vi "Project Save As.vi"(8 "error in (no error)":errorcluster, 9 "Rename Paths[]":T1[](array[typedef]), 10 "Existing Project Path":path, 11 "New Project Path":path) -> (0 "error out":errorcluster)   [LabVIEW 2016, in "SLL Scripting.lvlib"]
doc: "Make a copy of the project and rename some of the components of the project including their relinking."
uses:
  SLL Scripting.lvlib
  _Typedefs/Rename Item Cluster.ctl
  <vilib>/Utility/EditLVProj/Edit LVProj.lvlib
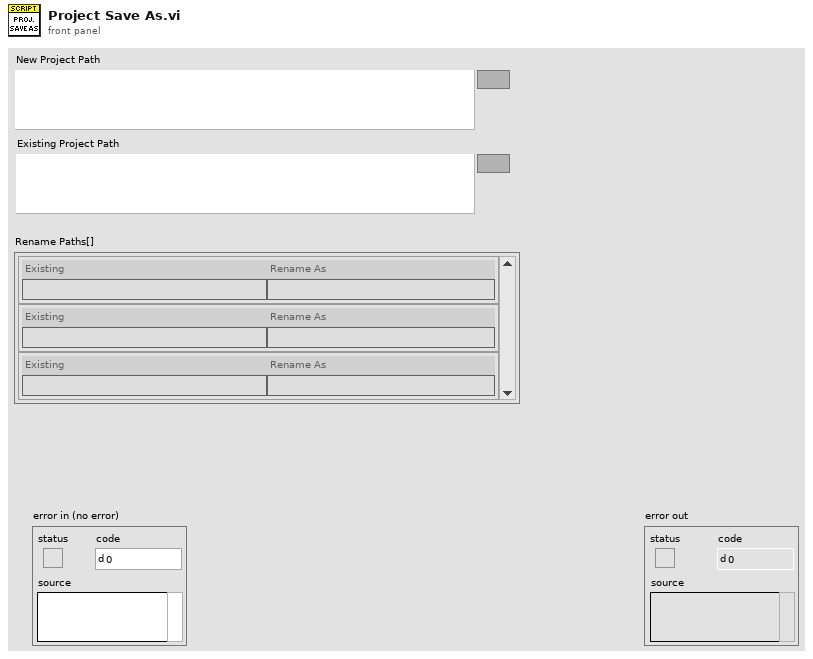
[diagram p1: front panel]
types:
  T1 = typedef "SLL Scripting.lvlib/Rename Item Cluster.ctl" = cluster{"Existing":string, "Rename As":string}
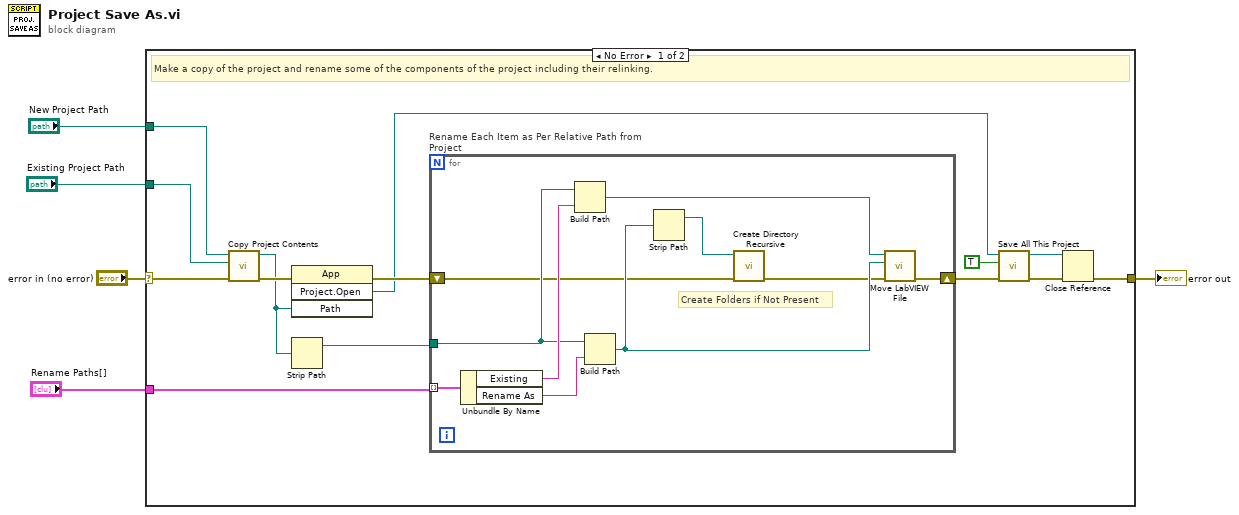
[diagram p0: block diagram]
diagram:
  n1 = case shown="No Error" "error in (no error)" {
    selector: "error in (no error)" -> [w19 w30]
    tunnel: [w8 w30] -> w4
    tunnel: "Existing Project Path" -> [w17 _]
    tunnel: "New Project Path" -> [w18 _]
    tunnel: "Rename Paths[]" -> [w14 _]
    frame No Error {
      # "Make a copy of the project and rename some of the components of the project including their relinking."
      n2 = call "Copy Project Contents.vi"("error in (no error)"=w19, "Existing Project Path"=w17, "New Project Path"=w18) -> ("error out"=w16:errorcluster, "New Project Path Out"=w13:path)  [unwired: 7 in]
      n3 = invoke class="App" method="Project.Open"(error in=w16, "Path"=w13) -> (error out=w15:errorcluster, "Project:Open"=w9:refnum<vi>)  [unwired: 2 in, 2 out]
      n4 = Strip Path(path=w13) -> (stripped path=w12:path)  [unwired: 1 out]
      n5 = for "Rename Each Item as Per Relative Path from Project" {
        shift-right: [w24] -> w11
        shift-left: w15 -> [w22]
        tunnel: w14 -> [w29] mode=indexing
        tunnel: w12 -> [w27]
        # "Create Folders if Not Present"
        n6 = Unbundle By Name(w29) -> ("Existing"=w28:string, "Rename As"=w26:string)
        n7 = Build Path(base path=w27, name or relative path=w28) -> (appended path=w25:path)
        n8 = Build Path(base path=w27, name or relative path=w26) -> (appended path=w23:path)
        n9 = Strip Path(path=w23) -> (stripped path=w20:path)  [unwired: 1 out]
        n10 = call <vilib>:"Create Directory Recursive.vi"("error in (no error)"=w22, "directory"=w20) -> ("error out"=w21:errorcluster)  [unwired: 3 in, 2 out]
        n11 = call "Move LabVIEW File.vi"("error in (no error)"=w21, "New Path"=w23, "Existing Path"=w25) -> ("error out"=w24:errorcluster)  [unwired: 8 in]
      }
      n12 = call <vilib>:"Save All This Project.vi"("error in (no error)"=w11, "Exclude Dependencies? (F)"=TRUE, "Project in"=w9) -> ("error out"=w10:errorcluster, "Project out"=w7:refnum<vi>)  [unwired: 7 in]
      n13 = Close Reference(reference=w7, error in (no error)=w10) -> (error out=w8:errorcluster)
    }
    frame Error {
    }
  }
  "error out" <- w4
